vi "Test MQTT-3.8.3-3.vi"(8 "error in (no error)":errorcluster, 11 "Connection Config":refnum<class "Connection.lvclass">) -> (0 "error out":errorcluster, 3 "Connection Config dup":refnum<class "Connection.lvclass">)   [LabVIEW 2013]
uses:
  <vilib>/LabVIEW Open Source Project/MQTT Connection/MQTT_Connection/Connection/Connection.lvclass
  <vilib>/LabVIEW Open Source Project/MQTT Control Packets/Control Packets/SUBSCRIBE/Topic Subscription -- cluster.ctl
  <vilib>/LabVIEW Open Source Project/MQTT Control Packets/Control Packets/ControlPacket/QualityOfService -- enum.ctl
  <vilib>/LabVIEW Open Source Project/MQTT Control Packets/Control Packets/ControlPacket/ControlPacket.lvclass/ControlPacket.ctl
  <vilib>/addons/_JKI Toolkits/Caraya/classes/Test/Test.lvclass
  <vilib>/LabVIEW Open Source Project/MQTT Client/Client class/Client.lvclass
  <vilib>/LabVIEW Open Source Project/MQTT Control Packets/Control Packets/SUBSCRIBE/SUBSCRIBE.lvclass
  <vilib>/addons/_JKI Toolkits/Caraya/classes/Assert/Assert.lvclass
  <vilib>/LabVIEW Open Source Project/MQTT Control Packets/Control Packets/ControlPacket/ControlPacket.lvclass
  <vilib>/LabVIEW Open Source Project/MQTT Connection/MQTT_Base/Base Class/MQTT_Base.lvclass
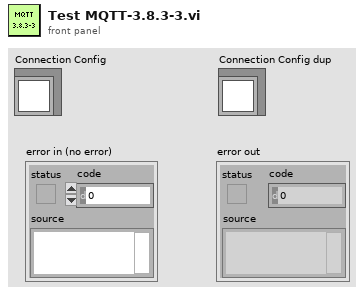
[diagram p1: front panel]
types:
  T1 = typedef "MQTT_Control_Packets.lvlib/SUBSCRIBE.lvclass/Topic Subscription -- cluster.ctl" = cluster{"Topic Filter":string, "QoS":T2}
  T2 = typedef "MQTT_Control_Packets.lvlib/ControlPacket.lvclass/QualityOfService -- enum.ctl" = enum16{"0 (At Most Once)", "1 (At Least Once)", "2 (Exactly Once)"}
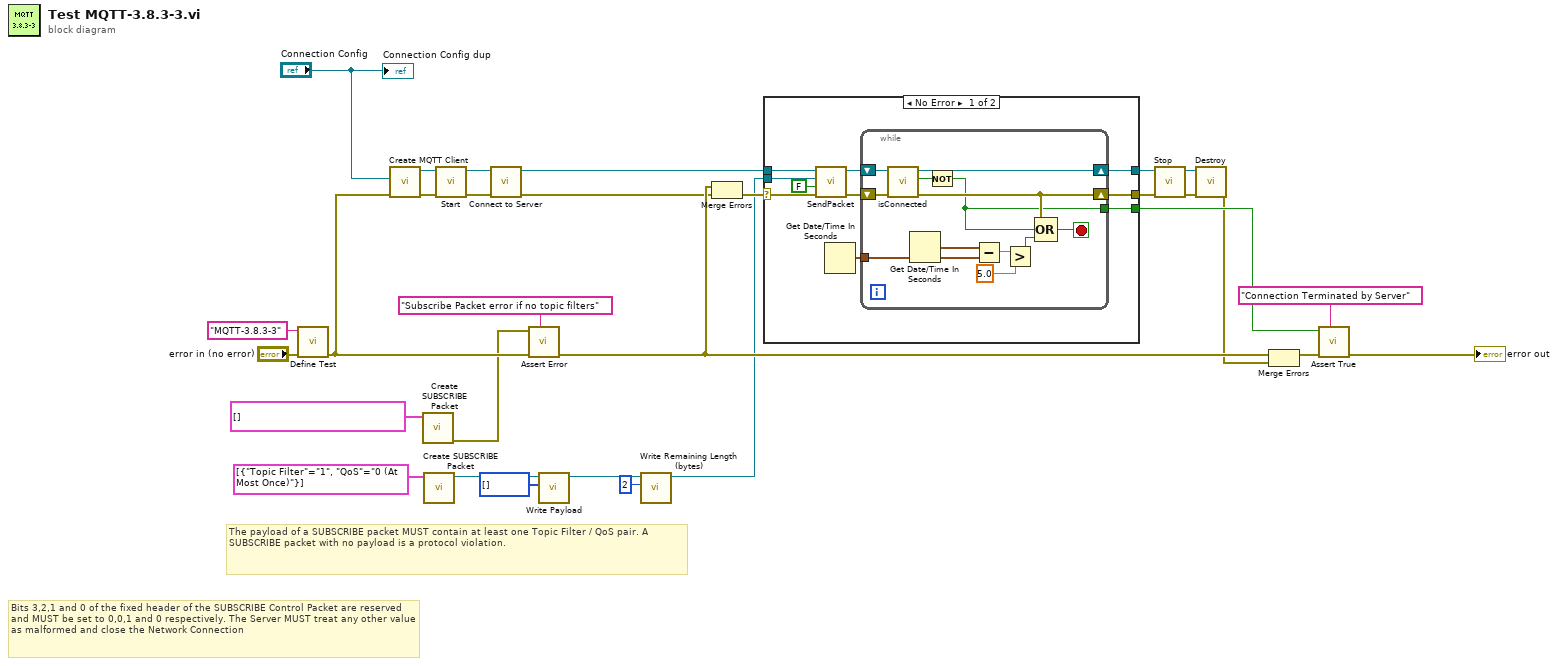
[diagram p0: block diagram]
diagram:
  # "The payload of a SUBSCRIBE packet MUST contain at least one Topic Filter / QoS pair. A SUBSCRIBE packet with no payload is a protocol violation."
  # "Bits 3,2,1 and 0 of the fixed header of the SUBSCRIBE Control Packet are reserved and MUST be set to 0,0,1 and 0 respectively. The Server MUST treat any other value as malformed and close the Network Connection"
  n1 = call <vilib>:"Define Test.vi"("error in (no error)"="error in (no error)", "Label (VI Title)"="MQTT-3.8.3-3") -> ("error out"=w23:errorcluster)  [unwired: 9 in]
  n2 = call <vilib>:"Create MQTT Client.vi"("error in (no error)"=w23, "Connection Configuration"="Connection Config") -> ("error out"=w15:errorcluster, "Client out"=w17:refnum<class "Client.lvclass">)  [unwired: 8 in]
  n3 = call <vilib>:"Create SUBSCRIBE Packet.vi"("Topic Subscriptions"=T1[] []) -> ("error out"=w13:errorcluster)  [unwired: 8 in, 2 out]
  n4 = call <vilib>:"Create SUBSCRIBE Packet.vi"("Topic Subscriptions"=T1[] [{"Topic Filter"="1", "QoS"=enum."0 (At Most Once)"}]) -> ("SUBSCRIBE out"=w11:refnum<class "SUBSCRIBE.lvclass">)  [unwired: 8 in, 2 out]
  n5 = call <vilib>:"Start.vi"("error in (no error)"=w15, "MQTT_Base in"=w17) -> ("error out"=w14:errorcluster, "MQTT_Base out"=w16:refnum<class "Client.lvclass">)  [unwired: 7 in, 1 out]
  n6 = call <vilib>:"Connect to Server.vi"("error in (no error)"=w14, "Client in"=w16) -> ("error out"=w19:errorcluster, "Client out"=w18:refnum<class "Client.lvclass">)  [unwired: 6 in, 2 out]
  n7 = call <vilib>:"Assert Error.vi"("Label"="Subscribe Packet error if no topic filters", "error in (no error)"=w23, "Error?"=w13) -> ("error out"=w21:errorcluster)  [unwired: 8 in]
  n8 = call <vilib>:"Write Payload.vi"("Payload"=u8[] [], "ControlPacket in"=w11) -> ("ControlPacket out"=w7:refnum<class "SUBSCRIBE.lvclass">)  [unwired: 9 in]
  n9 = call <vilib>:"Write Remaining Length (bytes).vi"("Remaining Length (bytes)"=u32 2, "ControlPacket in"=w7) -> ("ControlPacket out"=w9:refnum<class "SUBSCRIBE.lvclass">)  [unwired: 9 in]
  n10 = Merge Errors(w21, w19) -> (w20:errorcluster)
  n11 = case shown="No Error" w20 {
    selector: w20 -> [w39 _]
    tunnel: w18 -> [w40 w53]
    tunnel: [w33 _] -> w3
    tunnel: [w35 _] -> w26
    tunnel: w9 -> [w38 _]
    tunnel: [w32 w53] -> w5
    frame No Error {
      n12 = call <vilib>:"SendPacket.vi"("error in (no error)"=w39, "Wait for ack? (T)"=FALSE, "ControlPacket"=w38, "Client in"=w40) -> ("error out"=w36:errorcluster, "Client out"=w37:refnum<class "Client.lvclass">)  [unwired: 5 in, 1 out]
      n13 = Get Date/Time In Seconds() -> (seconds since 1Jan1904=w34:timestamp)
      n14 = while {
        shift-right: [w49] -> w33
        shift-left: w36 -> [w50]
        shift-right: [w51] -> w32
        shift-left: w37 -> [w52]
        tunnel: [w46] -> w35
        tunnel: w34 -> [w41]
        stop <- w48 stop-if-true
        n15 = call <vilib>:"isConnected.vi"("error in (no error)"=w50, "Client in"=w52) -> ("error out"=w49:errorcluster, "connected"=w47:bool, "Client out"=w51:refnum<class "Client.lvclass">)  [unwired: 7 in]
        n16 = Get Date/Time In Seconds() -> (seconds since 1Jan1904=w42:timestamp)
        n17 = Not(x=w47) -> (.not. x?=w46:bool)
        n18 = Subtract(x=w42, y=w41) -> (x-y=w45:dbl)
        n19 = Greater?(x=w45, y=5.0) -> (0:w43:bool)
        n20 = Compound Arithmetic op=OR(w49, w46, w43) -> (w48:bool)
      }
    }
    frame Error {
    }
  }
  n21 = call <vilib>:"Stop.vi"("error in (no error)"=w3, "MQTT_Base in"=w5) -> ("error out"=w2:errorcluster, "MQTT_Base out"=w6:refnum<class "Client.lvclass">)  [unwired: 7 in, 1 out]
  n22 = call <vilib>:"Destroy.vi"("error in (no error)"=w2, "MQTT_Base in"=w6) -> ("error out"=w4:errorcluster)  [unwired: 8 in, 1 out]
  n23 = Merge Errors(w21, w4) -> (w22:errorcluster)
  n24 = call <vilib>:"Assert True.vi"("Label"="Connection Terminated by Server", "error in (no error)"=w22, "True?"=w26) -> ("error out"=→"error out":errorcluster)  [unwired: 8 in]
  "Connection Config dup" <- "Connection Config"
